vi "Own20261012_CreateControlReference.vi"() -> ()   [LabVIEW 2024]
panel:
  out "error out":errorcluster caption="错误输出"
  out "reference_constant_id":refnum<vi>
  in  "control_id":u32
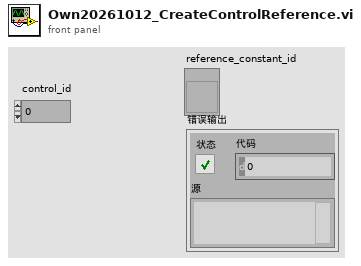
[diagram p1: front panel]
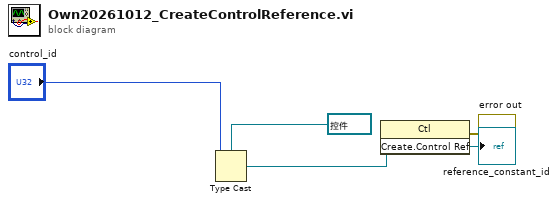
[diagram p0: block diagram]
diagram:
  n1 = Type Cast(type=refnum<vi> refnum ("引用"), x="control_id") -> (*(type *) &x=w3:refnum<vi>)
  n2 = invoke class="Ctl" method="Create.Control Ref"(reference=w3) -> (error out=→"error out":errorcluster, "Create Control Ref"=→"reference_constant_id":refnum<vi>)  [unwired: 2 in, 1 out]
